vi "Video Processing.vi"() -> ()   [LabVIEW 2014]
uses:
  AR.Drone 2.0 - Phase 4 - Auto hover above object with Video&Navdata method/AR Drone - Simple Video + Simple nav Folder/Global.vi
panel:
  in  "limit":sgl
  out "Vector sum Comp 1":dbl(slide) scale=-5.0..5.0
  out "Vector avg Comp 2":dbl(slide) scale=-5.0..5.0
  in  "Rectangle to ROI Extension":dbl=50.0 format="%#_13g"
  out "OF Video Out":T1(plugin-control)
  out "error out 2":errorcluster
  out "OF refresh":u32
  in  "Threshold":dbl(slide)=1.0 scale=0.0..20.0
  out "Video Loop":errorcluster
  out "Number of Particles before":i32
  out "Number of Particles after":i32
  in  "Number of Erosion":i32=30
  out "Video refresh":u32=48
  out "Read Video":errorcluster
  in  "milliseconds to wait":u32
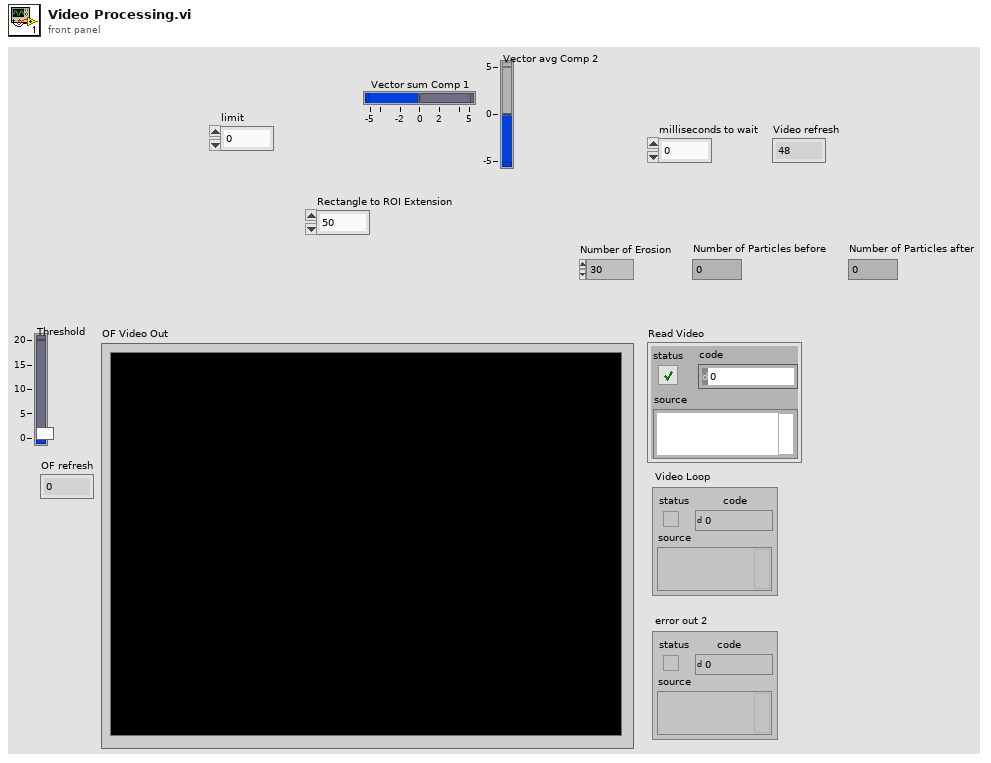
[diagram p1: front panel]
types:
  T1 = typedef "IMAQ Image.ctl" = refnum<image>
  T2 = cluster{"New Image":T1, "New Image":T1, "New Image":T1}
  T3 = typedef "ROI Descriptor" = cluster{"Global Rectangle":i32[], "Contours":cluster{"ID":enum32{"External", "Internal"}, "Type":u32, "Coordinates":i32[]}[]}
  T4 = cluster{"Numeric":dbl, "Numeric":dbl, "Numeric":dbl, "Numeric":dbl}
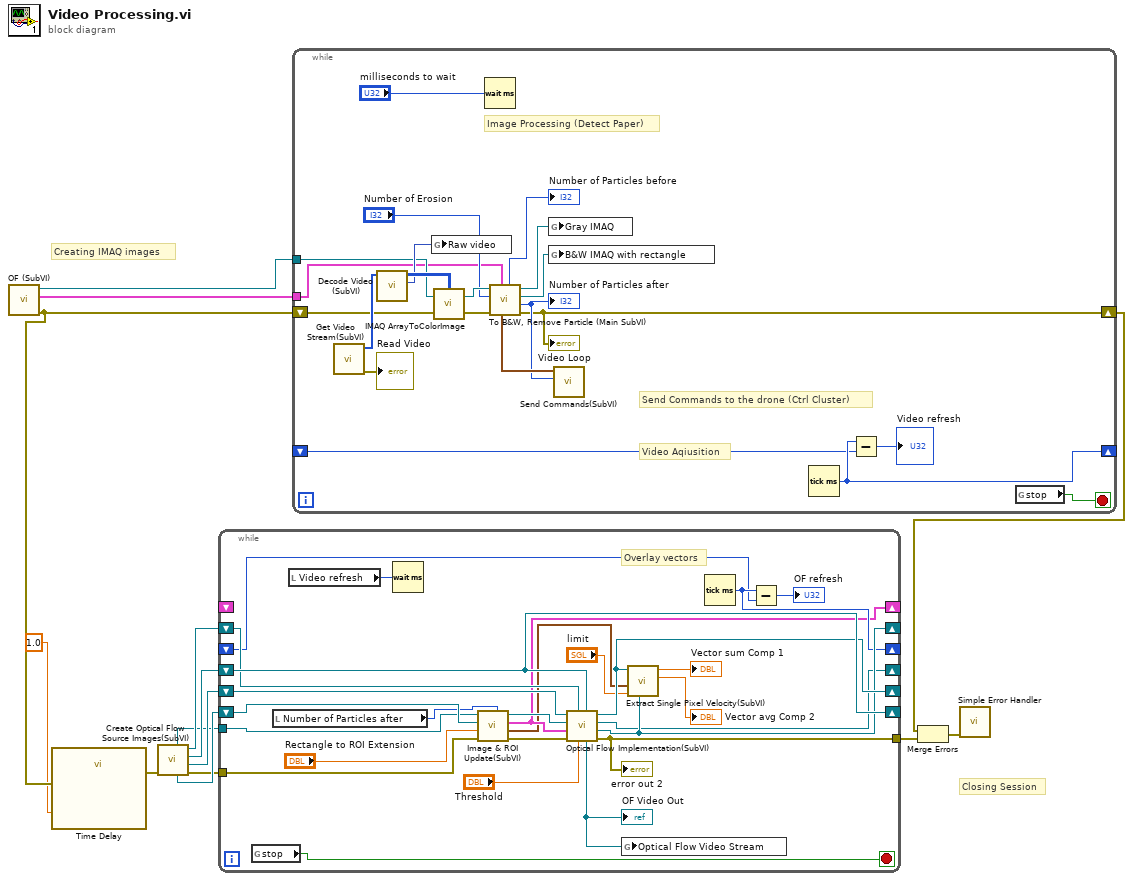
[diagram p0: block diagram]
diagram:
  # "Closing Session"
  # "Creating IMAQ images"
  n1 = call "OF (SubVI).vi"() -> ("error out"=w2:errorcluster, "Cluster"=w13:T2, "Refnum out"=w14:T1)  [unwired: 9 in]
  n2 = call "Time Delay"("error in (no error)"=w2, "Delay Time (s)"=1.0) -> ("error out"=w3:errorcluster)  [unwired: 9 in]
  n3 = call "Create Optical Flow Source Images(SubVI).vi"("error in (no error)"=w3) -> ("error out"=w9:errorcluster, "Optical Flow Velocity X"=w7:T1, "Optical Flow Previous Image"=w8:T1, "Optical Flow Velocity Y"=w6:T1, "Optical Flow Current Image"=w10:T1, "Raw input"=w5:T1)  [unwired: 5 in]
  n4 = while {
    shift-right: [w34] -> _
    shift-left: w7 -> [w39]
    shift-right: [w33] -> _
    shift-left: w6 -> [w38]
    shift-right: [w27] -> _
    shift-left: w8 -> [w40]
    shift-right: [w40] -> _
    shift-left: w10 -> [w36]
    tunnel: w5 -> [w26]
    shift-right: [w32] -> _
    shift-left: _ -> [w31]
    shift-right: [w23] -> _
    shift-left: _ -> [_]
    tunnel: w9 -> [w25]
    tunnel: [w35] -> w4
    stop <- w24 stop-if-true
    # "Overlay vectors"
    n5 = global read "Global.vi" "stop"() -> (w24:bool)
    n6 = local read "Number of Particles after"() -> (w15:i32)
    n7 = local read "Video refresh"() -> (w21:u32)
    n8 = Wait (ms)(milliseconds to wait=w21) -> ()  [unwired: 1 out]
    n9 = call "Image & ROI Update(SubVI).vi"("Nr of Objects"=w15, "error in (no error)"=w25, "Numeric"="Rectangle to ROI Extension", "Optical Flow Previous Image"=w36, "Refnum in"=w26) -> ("error out"=w28:errorcluster, "Rectangle"=w20:cluster{dbl, dbl, dbl, dbl, dbl}, "ROI Descriptor"=w23:T3, "Refnum out"=w29:T1)  [unwired: 3 in]
    n10 = call "Optical Flow Implementation(SubVI).vi"("Image Out in"=w40, "Threshold"="Threshold", "Velocity Component 2 Out in"=w38, "error in (no error)"=w28, "ROI Descriptor"=w23, "Image Dst Out"=w29, "Refnum in"=w39) -> ("error out"=w35:errorcluster, "Velocity Component 2 Out out"=w33:T1, "Image Out out"=w27:T1, "Velocity Component 1 Out out"=w34:T1, "Image"=w18:T1)
    "OF Video Out" <- w18
    "error out 2" <- w35
    n11 = global write "Global.vi" "Optical Flow Video Stream"(w18) -> ()
    n12 = call "Extract Single Pixel Velocity(SubVI).vi"("Velocity Component 2"=w33, "limit"="limit", "Rectangle"=w20, "Velocity Component 1"=w34) -> ("Vector sum Comp 2"=→"Vector avg Comp 2":dbl, "Vector sum Comp 1"=→"Vector sum Comp 1":dbl)  [unwired: 6 in]
    n13 = Tick Count (ms)() -> (millisecond timer value=w32:u32)
    n14 = Subtract(x=w32, y=w31) -> (x-y=→"OF refresh":u32)
  }
  n15 = while {
    shift-right: [w57] -> _
    shift-left: _ -> [w56]
    tunnel: w14 -> [w45]
    tunnel: w13 -> [w44]
    shift-right: [w43] -> w12
    shift-left: w2 -> [w46]
    stop <- w47 stop-if-true
    # "Send Commands to the drone (Ctrl Cluster)"
    # "Image Processing (Detect Paper)"
    # "Video Aqiusition"
    n16 = call "Get Video Stream(SubVI).vi"() -> ("error out"=→"Read Video":errorcluster, "ImgData"=w60:u8[])  [unwired: 10 in]
    n17 = call "Decode Video (SubVI).vi"("ImgData"=w60) -> ("new picture"=w54:picture, "Array"=w58:u32[][])  [unwired: 9 in]
    n18 = global write "Global.vi" "Raw video"(w54) -> ()
    n19 = call "IMAQ ArrayToColorImage"("Image Pixels (U32)"=w58, "Image"=w45, "error in (no error)"=w46) -> ("Image Out"=w53:T1, "error out"=w52:errorcluster)  [unwired: 2 in]
    n20 = Wait (ms)(milliseconds to wait="milliseconds to wait") -> ()  [unwired: 1 out]
    n21 = call "To B&W, Remove Particle (Main SubVI).vi"("Image Reference Sources"=w44, "error in (no error)"=w52, "Number of Erosion"="Number of Erosion", "Refnum in"=w53) -> ("error out"=w43:errorcluster, "Number of Particles after"=w48:i32, "Image Out"=w42:T1, "Current Grayscale"=w41:T1, "Number of Particles before"=→"Number of Particles before":i32, "Cluster"=w50:T4)  [unwired: 1 in, 1 out]
    "Number of Particles after" <- w48
    "Video Loop" <- w43
    n22 = global write "Global.vi" "Gray IMAQ"(w41) -> ()
    n23 = global write "Global.vi" "B&W IMAQ with rectangle"(w42) -> ()
    n24 = call "Send Commands(SubVI).vi"("Number of Particles after"=w48, "Cluster"=w50) -> ()  [unwired: 10 in]
    n25 = Tick Count (ms)() -> (millisecond timer value=w57:u32)
    n26 = Subtract(x=w57, y=w56) -> (x-y=→"Video refresh":u32)
    n27 = global read "Global.vi" "stop"() -> (w47:bool)
  }
  n28 = Merge Errors(w12, w4) -> (w11:errorcluster)
  n29 = call <vilib>:"Simple Error Handler.vi"("error in (no error)"=w11) -> ()  [unwired: 4 in, 5 out]
